vi "Exp curve fitting.vi"(10 "Color":T1, 11 "x (volts)":dbl) -> (3 "y (Lux)":dbl)   [LabVIEW 2020]
uses:
  controls/Color --typedef.ctl
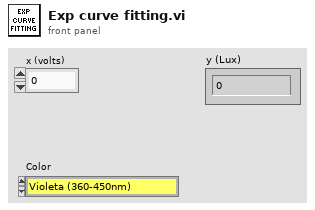
[diagram p1: front panel]
types:
  T1 = typedef "Color --typedef.ctl" = enum16{"Violeta (360-450nm)", "Azul (450-500nm)", "Verde(500-570nm)", "Amarillo (570-590nm)", "Naranja (600-610nm)", "Rojo (610-670nm)", "Blanco"}
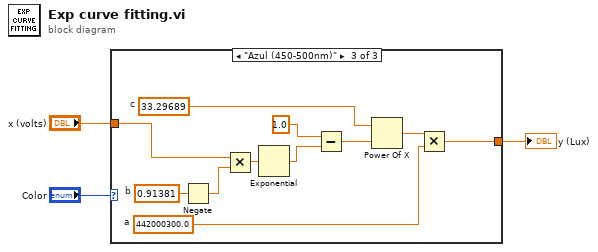
[diagram p0: block diagram]
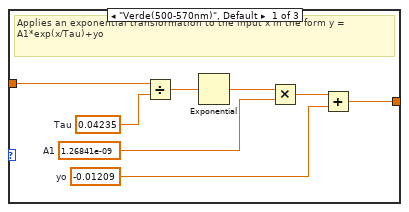
[diagram p2: hidden frame]
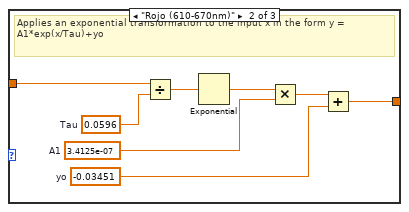
[diagram p3: hidden frame]
diagram:
  n1 = case shown="\"Azul (450-500nm)\"" "Color" {
    tunnel: "x (volts)" -> [w11 w19 w30]
    tunnel: [w4 w12 w20] -> w1
    frame "Verde(500-570nm)", Default {
      w7 = 1.26841e-09  # A1
      w5 = -0.01209  # yo
      w10 = 0.04235  # Tau
      # "Applies an exponential transformation to the input x in the form y = A1*exp(x/Tau)+yo"
      n2 = Divide(x=w11, y=w10) -> (x/y=w9:dbl)
      n3 = Exponential(1:w9) -> (0:w8:dbl)
      n4 = Multiply(x=w8, y=w7) -> (x*y=w6:dbl)
      n5 = Add(x=w6, y=w5) -> (x+y=w4:dbl)
    }
    frame "Rojo (610-670nm)" {
      w15 = 3.4125e-07  # A1
      w13 = -0.03451  # yo
      w18 = 0.0596  # Tau
      # "Applies an exponential transformation to the input x in the form y = A1*exp(x/Tau)+yo"
      n6 = Divide(x=w19, y=w18) -> (x/y=w17:dbl)
      n7 = Exponential(1:w17) -> (0:w16:dbl)
      n8 = Multiply(x=w16, y=w15) -> (x*y=w14:dbl)
      n9 = Add(x=w14, y=w13) -> (x+y=w12:dbl)
    }
    frame "Azul (450-500nm)" {
      w23 = 33.29689  # c
      w29 = 0.91381  # b
      w21 = 442000300.0  # a
      n10 = Negate(x=w29) -> (-x=w28:dbl)
      n11 = Multiply(x=w30, y=w28) -> (x*y=w27:dbl)
      n12 = Exponential(1:w27) -> (0:w26:dbl)
      n13 = Subtract(x=1.0, y=w26) -> (x-y=w24:dbl)
      n14 = Power Of X(1:w24, 2:w23) -> (0:w22:dbl)
      n15 = Multiply(x=w22, y=w21) -> (x*y=w20:dbl)
    }
  }
  "y (Lux)" <- w1
